vi "Test_Check_Groups_Caraya.vi"(8 "error in":errorcluster) -> (0 "error out":errorcluster)   [LabVIEW 2026]
doc: "Caraya tests for Evaluate Bool Group, Evaluate Range Group and Evaluate Compare Group, with chained asserts and one negative control restored."
uses:
  <vilib>/addons/_JKI Toolkits/Caraya/classes/Test/Test.lvclass
  <vilib>/addons/_JKI Toolkits/Caraya/classes/Assert/Assert.lvclass
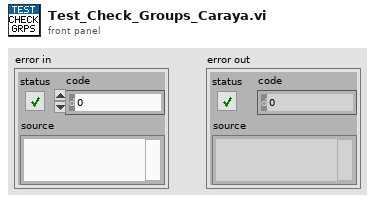
[diagram p1: front panel]
types:
  T1 = cluster{"name":string, "compare_with":string, "comparison":enum16{"EQ", "NE", "GT", "GE", "LT", "LE"}, "tolerance":dbl}[]
  T2 = cluster{"and_list":cluster{"name":string, "min":dbl, "max":dbl}[], "or_list":cluster{"name":string, "min":dbl, "max":dbl}[]}
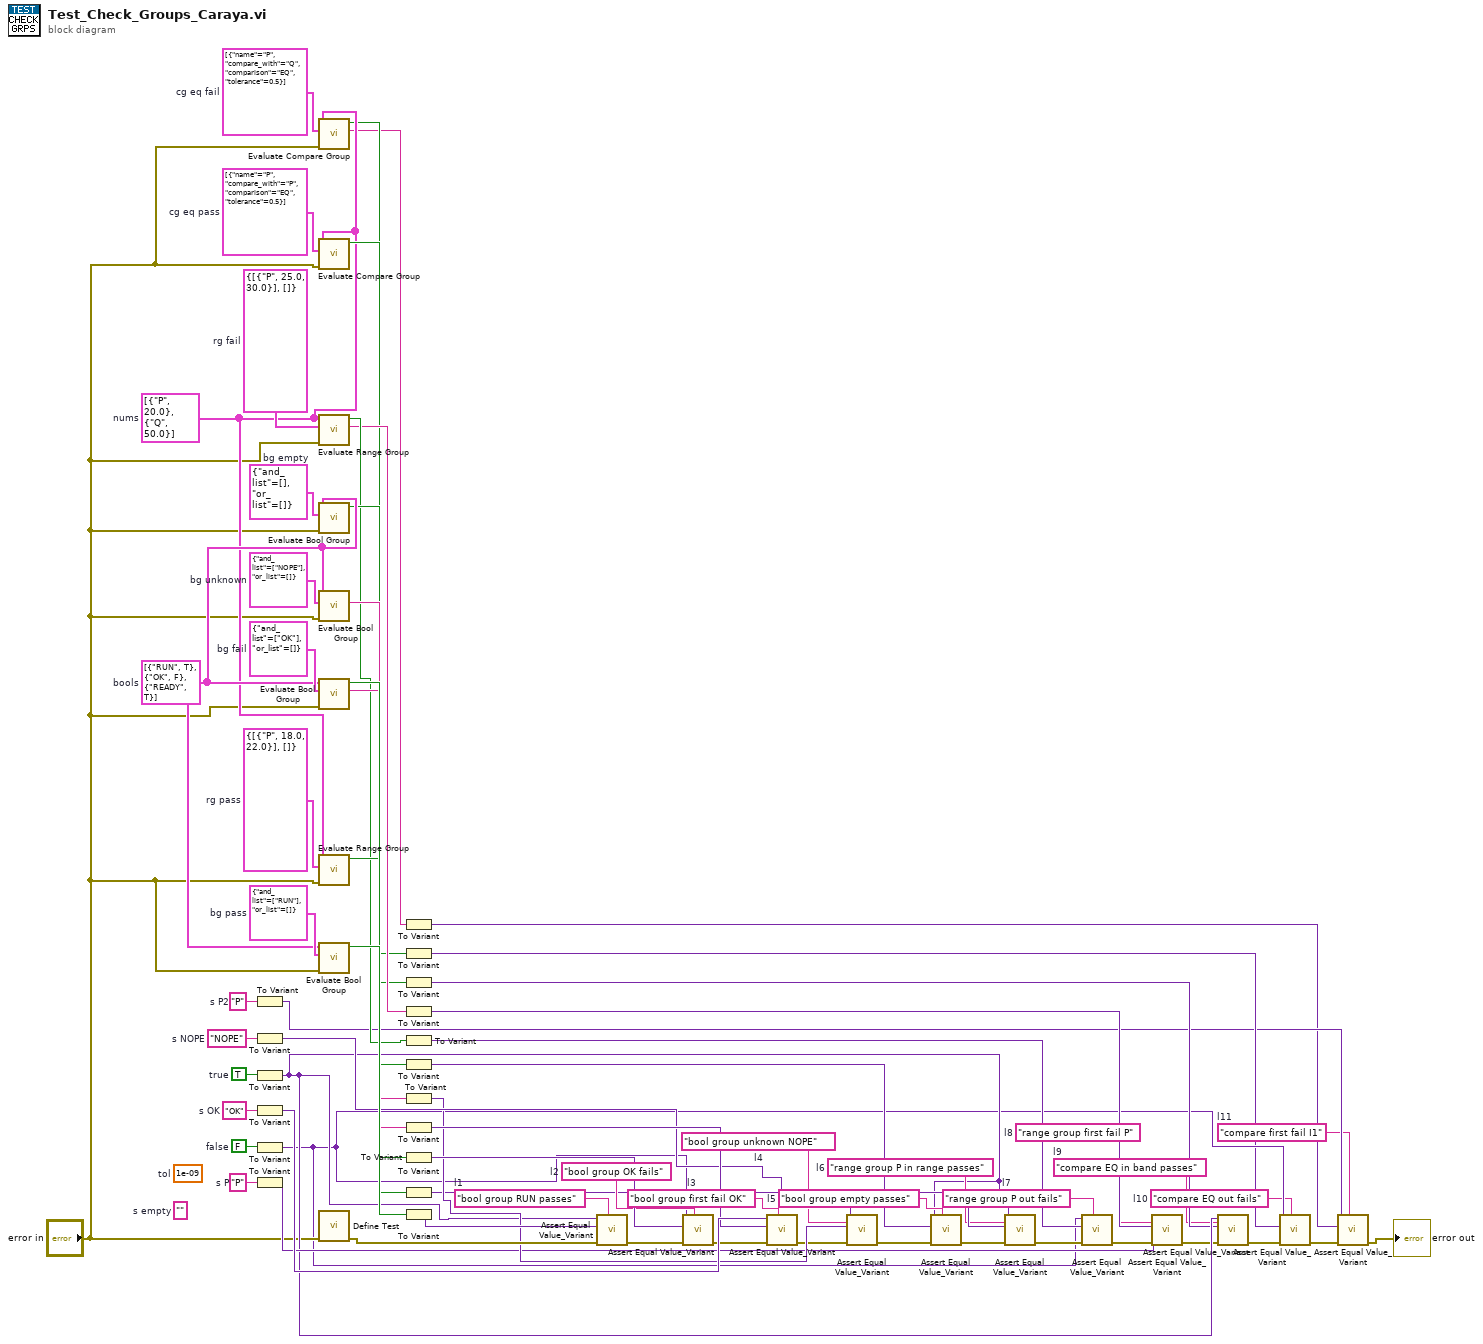
[diagram p0: block diagram]
diagram:
  w2 = "compare first fail I1"  # l11
  w8 = "compare EQ out fails"  # l10
  w16 = "compare EQ in band passes"  # l9
  w22 = "range group first fail P"  # l8
  w28 = "range group P out fails"  # l7
  w33 = "range group P in range passes"  # l6
  w38 = "bool group empty passes"  # l5
  w44 = "bool group unknown NOPE"  # l4
  w51 = "bool group first fail OK"  # l3
  w57 = "bool group OK fails"  # l2
  w63 = "bool group RUN passes"  # l1
  (unwired) 1e-09  # tol
  w6 = "P"  # s P2
  w26 = "P"  # s P
  w48 = "NOPE"  # s NOPE
  w55 = "OK"  # s OK
  (unwired) ""  # s empty
  w60 = FALSE  # false
  w66 = TRUE  # true
  w14 = T1 [{"name"="P", "compare_with"="Q", "comparison"=enum."EQ", "tolerance"=0.5}]  # cg eq fail
  w21 = T1 [{"name"="P", "compare_with"="P", "comparison"=enum."EQ", "tolerance"=0.5}]  # cg eq pass
  w32 = T2 {"and_list"=[{"name"="P", "min"=25.0, "max"=30.0}], "or_list"=[]}  # rg fail
  w37 = T2 {"and_list"=[{"name"="P", "min"=18.0, "max"=22.0}], "or_list"=[]}  # rg pass
  w42 = cluster{"and_list":string[], "or_list":string[]} {"and_list"=[], "or_list"=[]}  # bg empty
  w50 = cluster{"and_list":string[], "or_list":string[]} {"and_list"=["NOPE"], "or_list"=[]}  # bg unknown
  w62 = cluster{"and_list":string[], "or_list":string[]} {"and_list"=["OK"], "or_list"=[]}  # bg fail
  w68 = cluster{"and_list":string[], "or_list":string[]} {"and_list"=["RUN"], "or_list"=[]}  # bg pass
  w15 = cluster{"channel":string, "value":dbl}[] [{"channel"="P", "value"=20.0}, {"channel"="Q", "value"=50.0}]  # nums
  w43 = cluster{"name":string, "on":bool}[] [{"name"="RUN", "on"=TRUE}, {"name"="OK", "on"=FALSE}, {"name"="READY", "on"=TRUE}]  # bools
  n1 = To Variant(anything=w6) -> (Variant=w5:variant)
  n2 = To Variant(anything=w48) -> (Variant=w47:variant)
  n3 = To Variant(anything=w66) -> (Variant=w19:variant)
  n4 = To Variant(anything=w55) -> (Variant=w54:variant)
  n5 = To Variant(anything=w60) -> (Variant=w11:variant)
  n6 = To Variant(anything=w26) -> (Variant=w25:variant)
  n7 = call "Evaluate Compare Group.vi"("error in"="error in", "items"=w14, "num values"=w15) -> ("first fail"=w7:string, "passes"=w12:bool)  [unwired: 6 in, 1 out]
  n8 = call "Evaluate Compare Group.vi"("error in"="error in", "items"=w21, "num values"=w15) -> ("passes"=w20:bool)  [unwired: 6 in, 2 out]
  n9 = call "Evaluate Range Group.vi"("error in"="error in", "group"=w32, "num values"=w15) -> ("first fail"=w27:string, "passes"=w31:bool)  [unwired: 6 in, 1 out]
  n10 = call "Evaluate Bool Group.vi"("error in"="error in", "group"=w42, "bool values"=w43) -> ("passes"=w41:bool)  [unwired: 6 in, 2 out]
  n11 = call "Evaluate Bool Group.vi"("error in"="error in", "group"=w50, "bool values"=w43) -> ("first fail"=w49:string)  [unwired: 6 in, 2 out]
  n12 = call "Evaluate Bool Group.vi"("error in"="error in", "group"=w62, "bool values"=w43) -> ("first fail"=w56:string, "passes"=w61:bool)  [unwired: 6 in, 1 out]
  n13 = call "Evaluate Range Group.vi"("error in"="error in", "group"=w37, "num values"=w15) -> ("passes"=w36:bool)  [unwired: 6 in, 2 out]
  n14 = call "Evaluate Bool Group.vi"("error in"="error in", "group"=w68, "bool values"=w43) -> ("passes"=w67:bool)  [unwired: 6 in, 2 out]
  n15 = call <vilib>:"Define Test.vi"("error in (no error)"="error in") -> ("error out"=w64:errorcluster)  [unwired: 9 in, 1 out]
  n16 = To Variant(anything=w7) -> (Variant=w4:variant)
  n17 = To Variant(anything=w12) -> (Variant=w10:variant)
  n18 = To Variant(anything=w20) -> (Variant=w18:variant)
  n19 = To Variant(anything=w27) -> (Variant=w24:variant)
  n20 = To Variant(anything=w31) -> (Variant=w30:variant)
  n21 = To Variant(anything=w41) -> (Variant=w40:variant)
  n22 = To Variant(anything=w49) -> (Variant=w46:variant)
  n23 = To Variant(anything=w56) -> (Variant=w53:variant)
  n24 = To Variant(anything=w61) -> (Variant=w59:variant)
  n25 = To Variant(anything=w36) -> (Variant=w35:variant)
  n26 = To Variant(anything=w67) -> (Variant=w65:variant)
  n27 = call <vilib>:"Assert Equal Value_Variant.vi"("Label"=w63, "error in (no error)"=w64, "Actual"=w65, "Expected"=w19) -> ("error out"=w58:errorcluster)  [unwired: 6 in, 1 out]
  n28 = call <vilib>:"Assert Equal Value_Variant.vi"("Label"=w57, "error in (no error)"=w58, "Actual"=w59, "Expected"=w11) -> ("error out"=w52:errorcluster)  [unwired: 6 in, 1 out]
  n29 = call <vilib>:"Assert Equal Value_Variant.vi"("Label"=w51, "error in (no error)"=w52, "Actual"=w53, "Expected"=w54) -> ("error out"=w45:errorcluster)  [unwired: 6 in, 1 out]
  n30 = call <vilib>:"Assert Equal Value_Variant.vi"("Label"=w44, "error in (no error)"=w45, "Actual"=w46, "Expected"=w47) -> ("error out"=w39:errorcluster)  [unwired: 6 in, 1 out]
  n31 = call <vilib>:"Assert Equal Value_Variant.vi"("Label"=w38, "error in (no error)"=w39, "Actual"=w40, "Expected"=w19) -> ("error out"=w34:errorcluster)  [unwired: 6 in, 1 out]
  n32 = call <vilib>:"Assert Equal Value_Variant.vi"("Label"=w33, "error in (no error)"=w34, "Actual"=w35, "Expected"=w19) -> ("error out"=w29:errorcluster)  [unwired: 6 in, 1 out]
  n33 = call <vilib>:"Assert Equal Value_Variant.vi"("Label"=w28, "error in (no error)"=w29, "Actual"=w30, "Expected"=w11) -> ("error out"=w23:errorcluster)  [unwired: 6 in, 1 out]
  n34 = call <vilib>:"Assert Equal Value_Variant.vi"("Label"=w22, "error in (no error)"=w23, "Actual"=w24, "Expected"=w25) -> ("error out"=w17:errorcluster)  [unwired: 6 in, 1 out]
  n35 = call <vilib>:"Assert Equal Value_Variant.vi"("Label"=w16, "error in (no error)"=w17, "Actual"=w18, "Expected"=w19) -> ("error out"=w9:errorcluster)  [unwired: 6 in, 1 out]
  n36 = call <vilib>:"Assert Equal Value_Variant.vi"("Label"=w8, "error in (no error)"=w9, "Actual"=w10, "Expected"=w11) -> ("error out"=w3:errorcluster)  [unwired: 6 in, 1 out]
  n37 = call <vilib>:"Assert Equal Value_Variant.vi"("Label"=w2, "error in (no error)"=w3, "Actual"=w4, "Expected"=w5) -> ("error out"=→"error out":errorcluster)  [unwired: 6 in, 1 out]
